vi "LogicTrain-Sample-05-01-ALT.vi"() -> ()   [LabVIEW 2020]
uses:
  <vilib>/Rock Robotics/WPI/ThirdParty/JAS_Junk/TrajLib/Timer_New.vi
  <vilib>/Utility/semaphor.llb/Obtain Semaphore Reference.vi
  <vilib>/Rock Robotics/WPI/ThirdParty/JAS_Junk/TrajLib/Timer_Reset.vi
  <vilib>/Rock Robotics/WPI/ThirdParty/JAS_Junk/TrajLib/Timer_Start.vi
  <vilib>/Rock Robotics/WPI/ThirdParty/JAS_Junk/TrajLib/Timer_Stop.vi
  <vilib>/Rock Robotics/WPI/ThirdParty/JAS_Junk/TrajLib/Timer_HasPeriodPassedOnce.vi
  <vilib>/Rock Robotics/WPI/ThirdParty/JAS_Junk/TrajLib/Trajectory_Library.lvlib
panel:
  in  "Cancel Capture":bool
  out "Ready":bool
  out "Extend Arm":bool
  out "Close Hand":bool
  in  "Capture Cube":bool
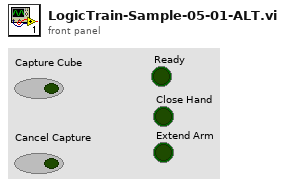
[diagram p1: front panel]
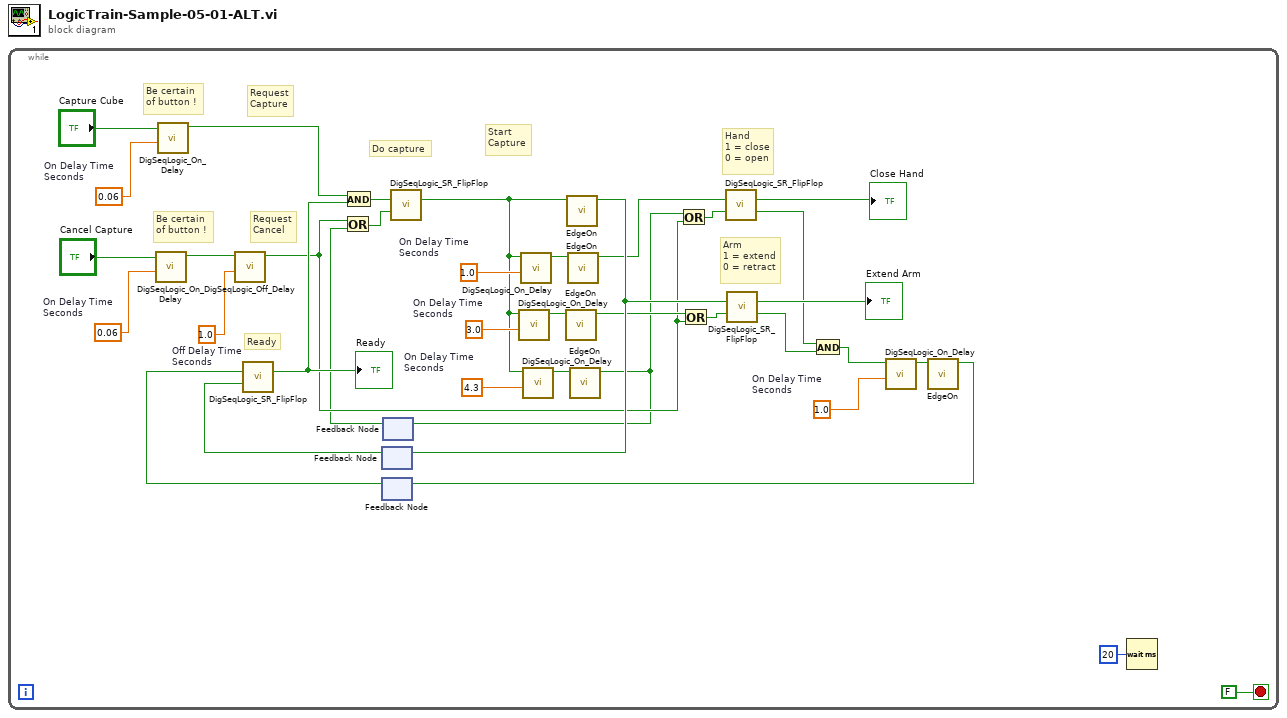
[diagram p0: block diagram]
diagram:
  n1 = while {
    stop <- FALSE stop-if-true
    w7 = 1.0  # Off Delay Time Seconds
    w15 = 0.06  # On Delay Time Seconds
    w29 = 4.3  # On Delay Time Seconds
    w31 = 3.0  # On Delay Time Seconds
    w33 = 1.0  # On Delay Time Seconds
    w36 = 0.06  # On Delay Time Seconds
    w37 = 1.0  # On Delay Time Seconds
    # "Request\nCapture"
    # "Request\nCancel"
    # "Be certain\nof button !"
    # "Do capture"
    # "Ready"
    # "Arm\n1 = extend\n0 = retract"
    # "Hand\n1 = close\n0 = open"
    # "Start\nCapture"
    # "Be certain\nof button !"
    n2 = call <vilib>:"DigSeqLogic_On_Delay.vi"("Delay"=w15, "Input"="Cancel Capture") -> ("Output"=w14:bool)  [unwired: 8 in, 1 out]
    n3 = call <vilib>:"DigSeqLogic_On_Delay.vi"("Delay"=w36, "Input"="Capture Cube") -> ("Output"=w34:bool)  [unwired: 8 in, 1 out]
    n4 = call <vilib>:"DigSeqLogic_Off_Delay.vi"("Delay"=w7, "Input"=w14) -> ("Output"=w4:bool)  [unwired: 8 in, 1 out]
    n5 = feedback #1() -> (w18:bool)  [unwired: 1 in]
    n6 = feedback #2() -> (w20:bool)  [unwired: 1 in]
    n7 = call <vilib>:"DigSeqLogic_SR_FlipFlop.vi"("Set"=w20, "Reset"=w18) -> ("Output"=w25:bool)  [unwired: 12 in, 1 out]
    "Ready" <- w25
    n8 = And(x=w34, y=w25) -> (x .and. y?=w6:bool)
    n9 = feedback #3() -> (w1:bool)  [unwired: 1 in]
    n10 = Or(x=w4, y=w1) -> (x .or. y?=w5:bool)
    n11 = call <vilib>:"DigSeqLogic_SR_FlipFlop.vi"("Set"=w6, "Reset"=w5) -> ("Output"=w12:bool)  [unwired: 12 in, 1 out]
    n12 = call <vilib>:"DigSeqLogic_On_Delay.vi"("Delay"=w31, "Input"=w12) -> ("Output"=w30:bool)  [unwired: 8 in, 1 out]
    n13 = call <vilib>:"DigSeqLogic_On_Delay.vi"("Delay"=w33, "Input"=w12) -> ("Output"=w32:bool)  [unwired: 8 in, 1 out]
    n14 = call <vilib>:"DigSeqLogic_On_Delay.vi"("Delay"=w29, "Input"=w12) -> ("Output"=w28:bool)  [unwired: 8 in, 1 out]
    n15 = call "EdgeOn.vi"("Input"=w30) -> ("Edge On"=w10:bool)  [unwired: 10 in]
    n16 = call "EdgeOn.vi"("Input"=w12) -> ("Edge On"=w19:bool)  [unwired: 10 in]
    n17 = feedback-in #1(w19) -> ()
    n18 = call "EdgeOn.vi"("Input"=w32) -> ("Edge On"=w13:bool)  [unwired: 10 in]
    n19 = call "EdgeOn.vi"("Input"=w28) -> ("Edge On"=w2:bool)  [unwired: 10 in]
    n20 = feedback-in #3(w2) -> ()
    n21 = Or(x=w2, y=w4) -> (x .or. y?=w9:bool)
    n22 = Or(x=w10, y=w4) -> (x .or. y?=w8:bool)
    n23 = call <vilib>:"DigSeqLogic_SR_FlipFlop.vi"("Set"=w13, "Reset"=w9) -> ("Output"=→"Close Hand":bool, "Inverse Output"=w24:bool)  [unwired: 12 in]
    n24 = call <vilib>:"DigSeqLogic_SR_FlipFlop.vi"("Set"=w19, "Reset"=w8) -> ("Output"=→"Extend Arm":bool, "Inverse Output"=w23:bool)  [unwired: 12 in]
    n25 = And(x=w24, y=w23) -> (x .and. y?=w22:bool)
    n26 = call <vilib>:"DigSeqLogic_On_Delay.vi"("Delay"=w37, "Input"=w22) -> ("Output"=w21:bool)  [unwired: 8 in, 1 out]
    n27 = call "EdgeOn.vi"("Input"=w21) -> ("Edge On"=w3:bool)  [unwired: 10 in]
    n28 = feedback-in #2(w3) -> ()
    n29 = Wait (ms)(milliseconds to wait=u32 20) -> ()  [unwired: 1 out]
  }
